vi "Panel.vi"(11 "AppListPanel in":refnum<class "AppListPanel.lvclass">) -> ()   [LabVIEW 2020, in "PicoG-App.lvlib" / "AppListPanel.lvclass"]
uses:
  AppListPanel.lvclass
  C:/Program Files (x86)/National Instruments/LabVIEW 2020/vi.lib/IlluminatedG/IG OOPanel/OOPanel/Panel/Panel.lvclass
  Sort Order.ctl
  <vilib>/IlluminatedG/IG OOPanel/OOPanel/Panel/Basic UI State.ctl
  AppListPanel.lvclass/AppListPanel.ctl
  GWebAppArrayPanel/GWebAppArrayPanel.lvclass
  C:/Program Files (x86)/National Instruments/LabVIEW 2020/vi.lib/IlluminatedG/IG OOPanel/OOPanel/ArrayPanel/ArrayPanel.lvclass
  ViaApp/ViaApp.lvclass
  <vilib>/IlluminatedG/IG OOPanel/OOPanel/Panel/Panel.lvclass
  <vilib>/IlluminatedG/IG OOPanel/OOPanel/OOPanel.lvlib
  <vilib>/IlluminatedG/IG OOPanel/OOPanel/ArrayManager/ArrayManager.lvclass
panel:
  in  "Sort Order":T1
  in  "Add":bool
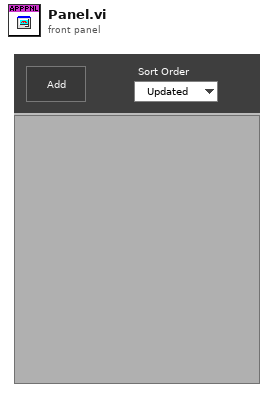
[diagram p1: front panel]
types:
  T1 = typedef "PicoG-App.lvlib/AppListPanel.lvclass/Sort Order.ctl" = enum16{"Updated", "Name"}
  T2 = typedef "OOPanel.lvlib/Panel.lvclass/Basic UI State.ctl" = enum16{"Init", "Run", "Close"}
  T3 = typedef "PicoG-App.lvlib/AppListPanel.lvclass/Inbound Events.ctl" = cluster{"Update App":refnum<user-event>, "Remove App":refnum<user-event>}
  T4 = typedef "OOPanel.lvlib/Panel.lvclass/Panel Events.ctl" = cluster{"Visbility":refnum<user-event>, "Close":refnum<user-event>}
  T5 = typedef "PicoG-App.lvlib/AppListPanel.lvclass/Ref Data.ctl" = cluster{"App Map":map{path, T6}}
  T6 = typedef "PicoG-App.lvlib/AppListPanel.lvclass/App Panel.ctl" = cluster{"App":refnum<class "ViaApp.lvclass">, "Panel":refnum<class "GWebAppArrayPanel.lvclass">}
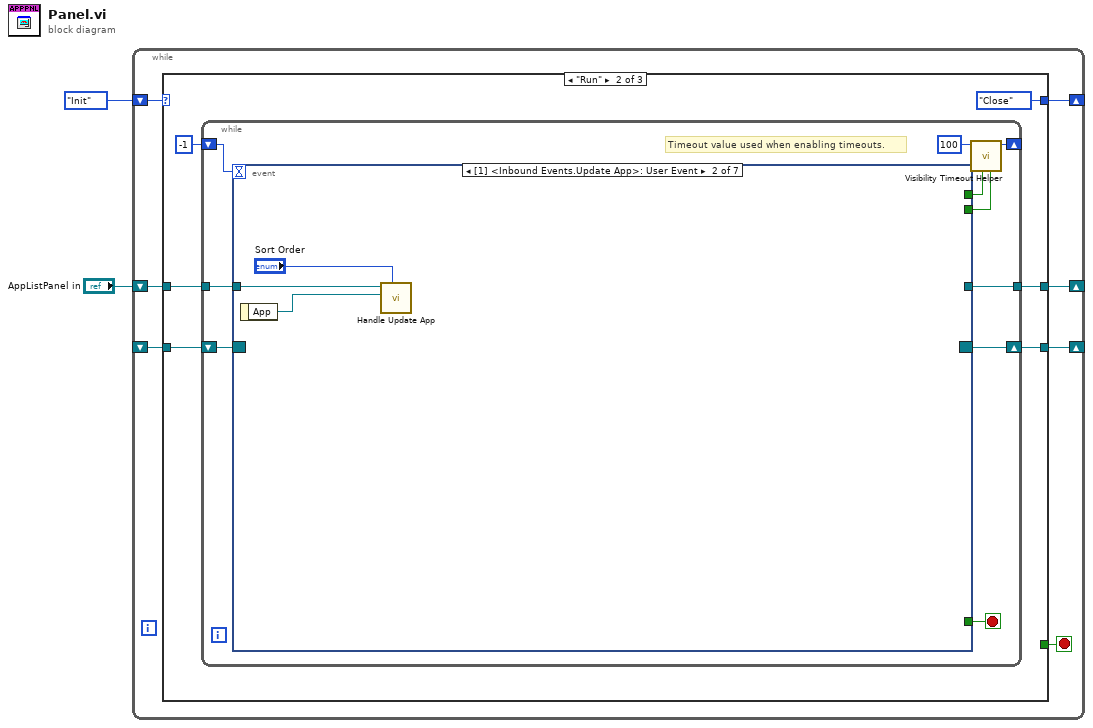
[diagram p0: block diagram]
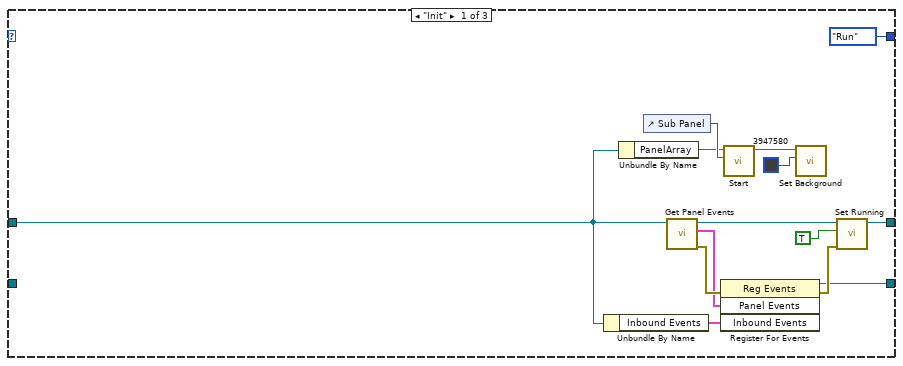
[diagram p2: hidden frame]
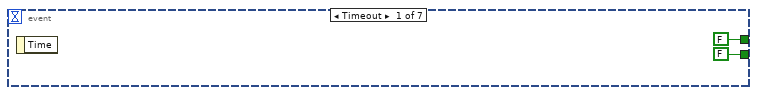
[diagram p3: hidden frame]
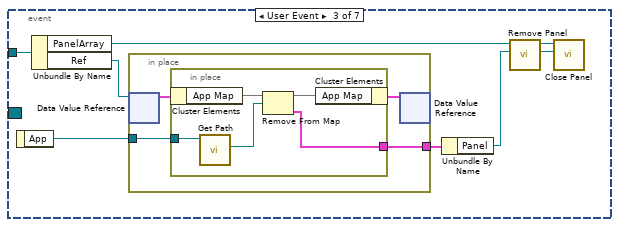
[diagram p4: hidden frame]
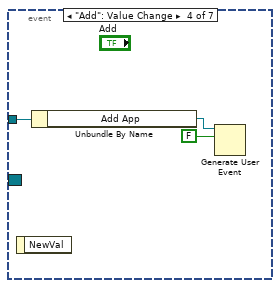
[diagram p5: hidden frame]
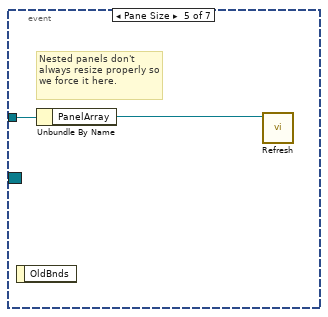
[diagram p6: hidden frame]
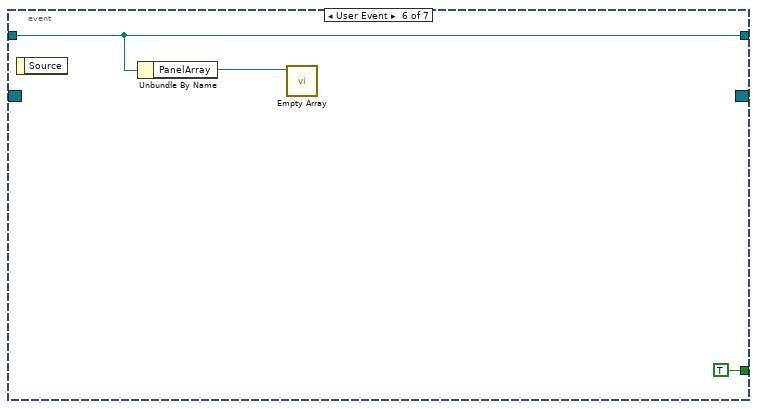
[diagram p7: hidden frame]
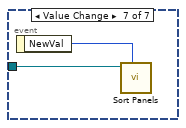
[diagram p8: hidden frame]
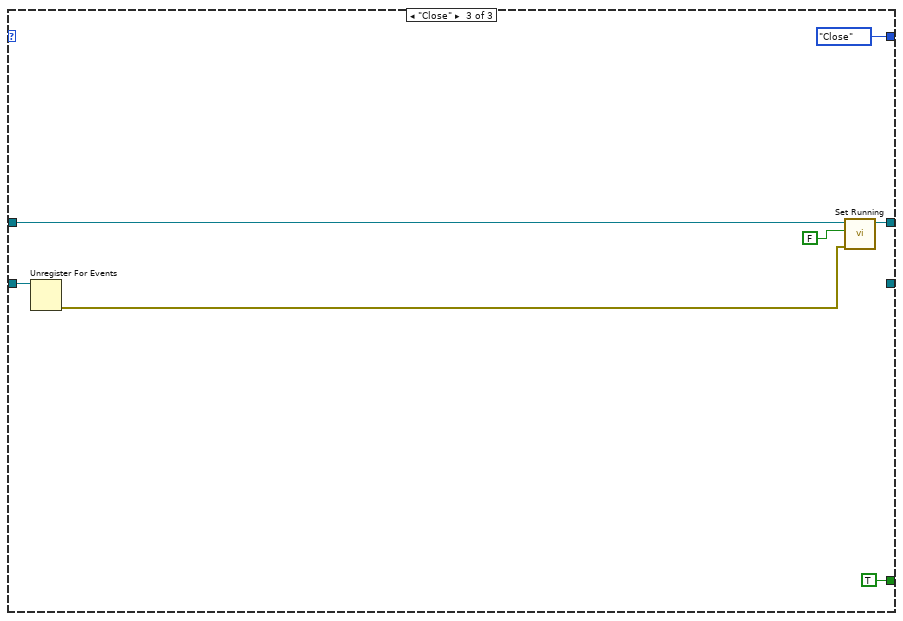
[diagram p9: hidden frame]
diagram:
  n1 = while {
    shift-right: [w8] -> _
    shift-left: _ -> [w9]
    shift-right: [w6] -> _
    shift-left: Basic_UI_State."Init" ("Basic UI State") -> [w7]
    shift-right: [w4] -> _
    shift-left: "AppListPanel in" -> [w3]
    stop <- w5 stop-if-true
    n2 = case shown="\"Run\"" w7 {
      tunnel: w9 -> [_ w29 w74]
      tunnel: [w17 w27 _] -> w8
      tunnel: [Basic_UI_State."Run" ("Basic UI State") Basic_UI_State."Close" ("Basic UI State") Basic_UI_State."Close" ("Basic UI State")] -> w6
      tunnel: [_ _ TRUE] -> w5
      tunnel: [w16 w24 w72] -> w4
      tunnel: w3 -> [w12 w25 w73]
      frame "Init" {
        n3 = Unbundle By Name(w12) -> ("Inbound Events"=w13:T3)
        n4 = Unbundle By Name(w12) -> ("PanelArray"=w14:refnum<class "ArrayManager.lvclass">)
        n5 = control-ref of="Sub Panel"() -> (w15:refnum<vi>)
        n6 = call <vilib>:"Get Panel Events.vi"("Panel in"=w12) -> ("error out"=w23:errorcluster, "Panel Events"=w19:T4, "Panel out"=w20:refnum<class "AppListPanel.lvclass">)  [unwired: 8 in]
        n7 = register-events(error in=w23, w19, w13) -> (reference out=w17:refnum<event-registration>, error out=w21:errorcluster)  [unwired: 1 in]
        n8 = call <vilib>:"Start.vi"("Container"=w15, "ArrayManager in"=w14) -> ("ArrayManager out"=w11:refnum<class "ArrayManager.lvclass">)  [unwired: 8 in, 1 out]
        n9 = call <vilib>:"Set Background.vi"("Background"=u32 3947580, "ArrayManager in"=w11) -> ()  [unwired: 8 in, 2 out]
        n10 = call <vilib>:"Set Running.vi"("error in (no error)"=w21, "Running"=TRUE, "Panel in"=w20) -> ("Panel out"=w16:refnum<class "AppListPanel.lvclass">)  [unwired: 7 in, 1 out]
      }
      frame "Run" {
        n11 = while {
          shift-right: [w35] -> w27
          shift-left: w29 -> [w36]
          shift-right: [w38] -> _
          shift-left: -1 ("Timeout") -> [w37]
          tunnel: w25 -> [w31]
          tunnel: [w30] -> w24
          stop <- w32 stop-if-true
          # "Timeout value used when enabling timeouts."
          n12 = event shown="[1] <Inbound Events.Update App>: User Event" {
            selector: w36 -> [_ _ _ _ _ _ _]
            dyn-events: [_ _ _ _ _ _ _] -> w35
            timeout: w37 -> [_ _ _ _ _ _ _]
            tunnel: [FALSE _ _ _ _ _ _] -> w34
            tunnel: [FALSE _ _ _ _ _ _] -> w33
            tunnel: [_ _ _ _ _ TRUE _] -> w32
            tunnel: w31 -> [_ w44 w51 w64 w66 w68 w70]
            tunnel: [_ _ _ _ _ w68 _] -> w30
            event Timeout {
              n13 = event-data() -> ()  [unwired: 1 in, 1 out]
            }
            event User Event {
              n14 = event-data() -> ("App"=w43:refnum<class "ViaApp.lvclass">)  [unwired: 1 in]
              n15 = call "Handle Update App.vi"("Sort Order"="Sort Order", "ViaApp"=w43, "AppListPanel in"=w44) -> ()  [unwired: 7 in, 2 out]
            }
            event User Event {
              n16 = event-data() -> ("App"=w50:refnum<class "ViaApp.lvclass">)  [unwired: 1 in]
              n17 = Unbundle By Name(w51) -> ("PanelArray"=w48:refnum<class "ArrayManager.lvclass">, "Ref"=w52:refnum<data-value>)
              n18 = in-place {
                in-place-border: w50 -> [w54]
                in-place-border: [w53] -> w49
                n19 = in-place-dvr #1(w52) -> (w56:T5)  [unwired: 1 out]
                n20 = in-place {
                  in-place-border: w54 -> [w61]
                  in-place-border: [w57] -> w53
                  n21 = in-place-cluster #2(w56) -> ("App Map"=w60:map{path, T6})
                  n22 = call "Get Path.vi"("ViaApp in"=w61) -> ("Path"=w59:path)  [unwired: 8 in, 2 out]
                  n23 = Remove From Map(10:w59, 11:w60) -> (1:w57:T6, 3:w58:map{path, T6})  [unwired: 1 out]
                  n24 = in-place-cluster #2("App Map"=w58) -> (w55:T5)
                }
                n25 = in-place-dvr #1(w55) -> ()  [unwired: 2 out]
              }
              n26 = Unbundle By Name(w49) -> ("Panel"=w47:refnum<class "GWebAppArrayPanel.lvclass">)
              n27 = call <vilib>:"Remove Panel.vi"("Panel in"=w47, "ArrayManager in"=w48) -> ("Panel"=w45:refnum<class "ArrayPanel.lvclass">, "ArrayManager out"=w46:refnum<class "ArrayManager.lvclass">)  [unwired: 7 in, 1 out]
              n28 = call <vilib>:"Close Panel.vi"("ArrayPanel"=w45, "ArrayManager in"=w46) -> ()  [unwired: 8 in, 2 out]
            }
            event "Add": Value Change {
              n29 = event-data() -> ()  [unwired: 1 in, 1 out]
              n30 = Unbundle By Name(w64) -> ("Add App"=w63:refnum<user-event>)
              n31 = Generate User Event(user event=w63, event data cluster=FALSE ("event data")) -> ()  [unwired: 2 in, 2 out]
            }
            event Pane Size {
              # "Nested panels don't always resize properly so we force it here."
              n32 = event-data() -> ()  [unwired: 1 in, 1 out]
              n33 = Unbundle By Name(w66) -> ("PanelArray"=w65:refnum<class "ArrayManager.lvclass">)
              n34 = call <vilib>:"Refresh.vi"("ArrayManager in"=w65) -> ()  [unwired: 9 in, 2 out]
            }
            event User Event {
              n35 = event-data() -> ()  [unwired: 1 in, 1 out]
              n36 = Unbundle By Name(w68) -> ("PanelArray"=w67:refnum<class "ArrayManager.lvclass">)
              n37 = call <vilib>:"Empty Array.vi"("ArrayManager in"=w67) -> ()  [unwired: 9 in, 2 out]
            }
            event Value Change {
              n38 = event-data() -> ("NewVal"=w71:T1)  [unwired: 1 in]
              n39 = call "Sort Panels.vi"("Sort Order"=w71, "AppListPanel"=w70) -> ()  [unwired: 9 in, 1 out]
            }
          }
          n40 = call <vilib>:"Visibility Timeout Helper.vi"("Update?"=w33, "Use Timeout?"=w34, "Visible Timeout mS"=100) -> ("Timeout"=w38:i32)  [unwired: 8 in]
        }
      }
      frame "Close" {
        n41 = Unregister For Events(event registration refnum=w74) -> (error out=w76:errorcluster)  [unwired: 1 in]
        n42 = call <vilib>:"Set Running.vi"("error in (no error)"=w76, "Running"=FALSE, "Panel in"=w73) -> ("Panel out"=w72:refnum<class "AppListPanel.lvclass">)  [unwired: 7 in, 1 out]
      }
    }
  }
